vi "Build Stream Object.vi"(10 "cancelled":refnum<queue>, 11 "events":refnum<queue>) -> (3 "stream":string)   [LabVIEW 2020, in "MCP Server.lvlib"]
doc: "Builds the stream object that Run Streamed Request.vi puts into the request context of a streamed tools/call: {\"events\":<n>,\"cancelled\":<m>}, where n and m are the two queue refnums of the MCP SSE Response as numbers. Get Request Stream.vi turns them back into queues, and the text identifies the stream (stream key)."
uses:
  MCP Server.lvlib
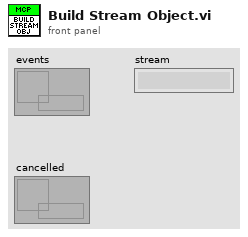
[diagram p1: front panel]
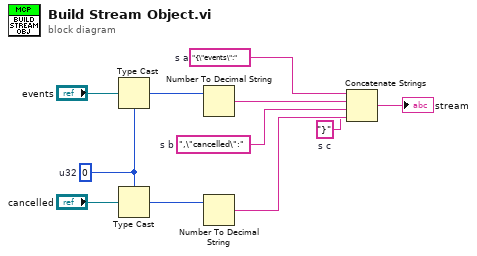
[diagram p0: block diagram]
diagram:
  w6 = "}"  # s c
  w5 = ",\"cancelled\":"  # s b
  w4 = "{\"events\":"  # s a
  w3 = u32 0  # u32
  n1 = Type Cast(type=w3, x="events") -> (*(type *) &x=w7:u32)
  n2 = Type Cast(type=w3, x="cancelled") -> (*(type *) &x=w8:u32)
  n3 = Number To Decimal String(number=w7) -> (decimal integer string=w9:string)  [unwired: 1 in]
  n4 = Number To Decimal String(number=w8) -> (decimal integer string=w10:string)  [unwired: 1 in]
  n5 = Concatenate Strings(w4, w9, w5, w10, w6) -> (→"stream":string)
